vi "OwnInterface20261013_Create.vi"() -> ()   [LabVIEW 2024]
uses:
  <resource>/Framework/Providers/AddInterface/Add Interface.lvlib
panel:
  out "error out":errorcluster caption="错误输出"
  in  "New Interface Owner":refnum<vi>
  in  "Parent Interfaces":refnum<vi>[](array[refnum])
  in  "Interface Path":path
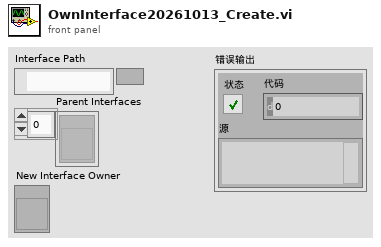
[diagram p1: front panel]
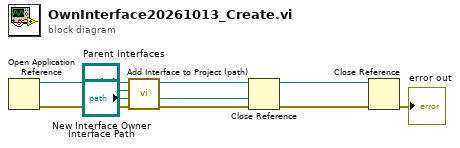
[diagram p0: block diagram]
diagram:
  n1 = Open Application Reference() -> (0:w8:errorcluster, 3:w9:refnum<vi>)  [unwired: 4 in]
  n2 = call <resource>:"Add Interface to Project (path).vi"("Application"=w9, "error in"=w8, "Interface Path"="Interface Path", "New Interface Owner"="New Interface Owner", "Parent Interfaces"="Parent Interfaces") -> ("error out"=w3:errorcluster, "Interface"=w4:refnum<vi>)  [unwired: 5 in]
  n3 = Close Reference(reference=w4, error in (no error)=w3) -> (error out=w2:errorcluster)
  n4 = Close Reference(reference=w9, error in (no error)=w2) -> (error out=→"error out":errorcluster)
